vi "VIH HelpGen - Get Nested Control Refnums.vi"(7 "Expand Tab Control (F)":bool, 8 "error in":errorcluster, 9 "Skip Cluster if it's Array element (T)":bool=TRUE, 10 "Get members (T)":bool=TRUE, 11 "Ctl Refnum":refnum<vi>) -> (0 "error out":errorcluster, 2 "Ctl Refnums":refnum<vi>[](array[refnum]), 3 "dup Ctl Refnum":refnum<vi>)   [LabVIEW 2014]
doc: "::: VI Helpeks :::\nCopyright (c) 2000-2026 Konstantin Shifershteyn. All rights reserved."
panel:
  # "VI Helpeks\nCopyright (c) 2012-2026 Konstantin Shifershteyn"
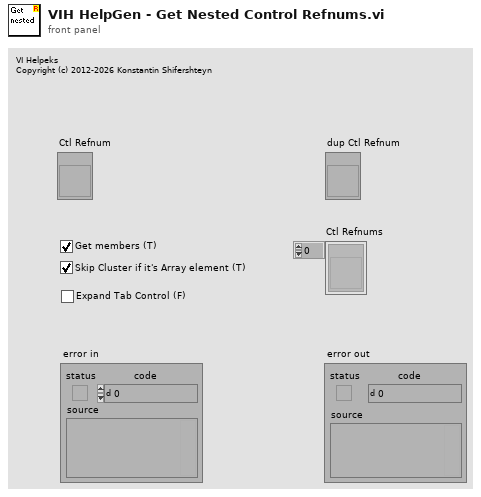
[diagram p1: front panel]
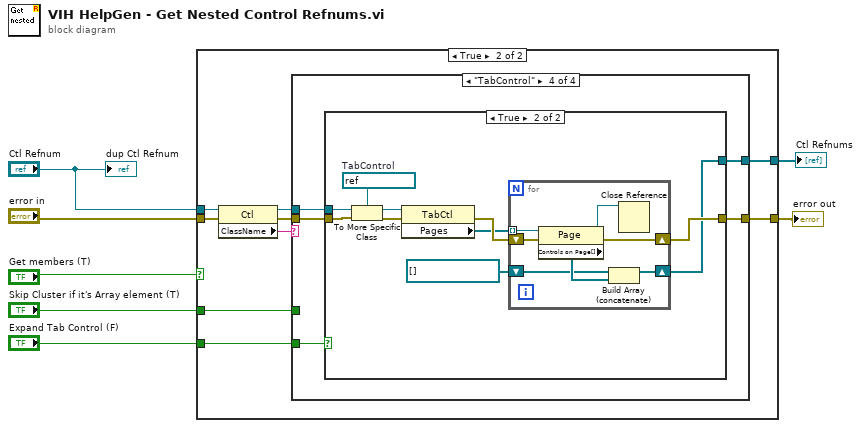
[diagram p0: block diagram]
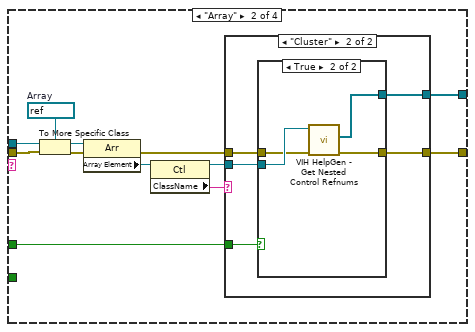
[diagram p4: hidden frame]
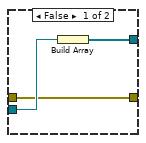
[diagram p6: hidden frame]
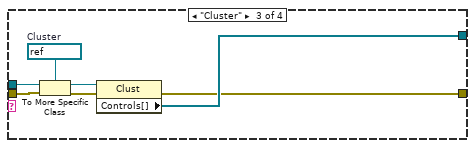
[diagram p7: hidden frame]
diagram:
  n1 = case shown="True" "Get members (T)" {
    tunnel: "Ctl Refnum" -> [_ w14]
    tunnel: "error in" -> [w8 w13]
    tunnel: [_ w12] -> w5
    tunnel: [w8 w11] -> w4
    tunnel: "Skip Cluster if it's Array element (T)" -> [_ w10]
    tunnel: "Expand Tab Control (F)" -> [_ w9]
    frame False {
    }
    frame True {
      n2 = property class="Ctl"(reference=w14, error in=w13) -> (reference out=w17:refnum<vi>, error out=w16:errorcluster, "ClassName"=w15:string)
      n3 = case shown="\"TabControl\"" w15 {
        tunnel: w17 -> [_ w30 w50 w55]
        tunnel: w16 -> [w18 w29 w49 w54]
        tunnel: [_ w28 w48 w52] -> w12
        tunnel: [w18 w20 w47 w53] -> w11
        tunnel: w10 -> [_ w19 _ _]
        tunnel: w9 -> [_ _ _ w51]
        frame Default {
        }
        frame "Array" {
          w25 = refnum<vi> refnum  # Array
          n4 = To More Specific Class(target class=w25, reference=w30, error in=w29) -> (specific class reference=w26:refnum<vi>, error out=w27:errorcluster)
          n5 = property class="Arr"(reference=w26, error in=w27) -> (error out=w21:errorcluster, "Array Element"=w24:refnum<vi>)  [unwired: 1 out]
          n6 = property class="Ctl"(reference=w24) -> (reference out=w23:refnum<vi>, "ClassName"=w22:string)  [unwired: 1 in, 1 out]
          n7 = case shown="\"Cluster\"" w22 {
            tunnel: [_ w36] -> w28
            tunnel: w23 -> [_ w35]
            tunnel: w21 -> [w31 w34]
            tunnel: [w31 w33] -> w20
            tunnel: w19 -> [_ w32]
            frame Default {
            }
            frame "Cluster" {
              n8 = case shown="True" w32 {
                tunnel: [w39 w42] -> w36
                tunnel: w35 -> [w38 w43]
                tunnel: w34 -> [w37 w41]
                tunnel: [w37 w40] -> w33
                frame False {
                  n9 = Build Array(w38) -> (w39:refnum<vi>[])
                }
                frame True {
                  n10 = call "VIH HelpGen - Get Nested Control Refnums.vi"("error in"=w41, "Ctl Refnum"=w43) -> ("error out"=w40:errorcluster, "Ctl Refnums"=w42:refnum<vi>[])  [unwired: 7 in, 1 out]
                }
              }
            }
          }
        }
        frame "Cluster" {
          w44 = refnum<vi> refnum  # Cluster
          n11 = To More Specific Class(target class=w44, reference=w50, error in=w49) -> (specific class reference=w45:refnum<vi>, error out=w46:errorcluster)
          n12 = property class="Clust"(reference=w45, error in=w46) -> (error out=w47:errorcluster, "Controls[]"=w48:refnum<vi>[])  [unwired: 1 out]
        }
        frame "TabControl" {
          n13 = case shown="True" w51 {
            tunnel: w55 -> [_ w60]
            tunnel: w54 -> [w56 w59]
            tunnel: [w56 w58] -> w53
            tunnel: [_ w57] -> w52
            frame False {
            }
            frame True {
              w61 = refnum<vi> refnum  # TabControl
              n14 = To More Specific Class(target class=w61, reference=w60, error in=w59) -> (specific class reference=w62:refnum<vi>, error out=w63:errorcluster)
              n15 = property class="TabCtl"(reference=w62, error in=w63) -> (error out=w65:errorcluster, "Pages"=w64:refnum<vi>[])  [unwired: 1 out]
              n16 = for {
                tunnel: w64 -> [w73] mode=indexing
                shift-right: [w71] -> w58
                shift-left: w65 -> [w72]
                shift-right: [w68] -> w57
                shift-left: refnum<vi>[] [] -> [w69]
                n17 = property class="Page"(reference=w73, error in=w72) -> (reference out=w67:refnum<vi>, error out=w71:errorcluster, "Controls on Page[]"=w70:refnum<vi>[])
                n18 = Build Array (concatenate)(w69, w70) -> (w68:refnum<vi>[])
                n19 = Close Reference(reference=w67) -> ()  [unwired: 1 in, 1 out]
              }
            }
          }
        }
      }
    }
  }
  "error out" <- w4
  "Ctl Refnums" <- w5
  "dup Ctl Refnum" <- "Ctl Refnum"
